vi "VIH Project Tree - Add Files.vi"(6 "Ena dialog message (F)":bool, 8 "error in":errorcluster, 9 "File Paths":path[](array[path]), 10 "Tree Parent Tag":string, 11 "Project Tree":T1) -> (0 "error out":errorcluster, 1 "Top-level Item Tags":string[](array[string]), 3 "dup Project Tree":T1, 4 "Files already in the tree":path[](array[path]))   [LabVIEW 2014]
doc: "::: VI Helpeks :::\nCopyright (c) 2000-2026 Konstantin Shifershteyn. All rights reserved."
uses:
  VIH Project Tree Typedef - Tree Refnum.ctl
  _VIH HelpGen - Palette.llb/VIH HelpGen Typedef - Palette - Item Info Cluster.ctl
  _VIH HelpGen - Palette.llb/VIH HelpGen Typedef - Palette - Item Type Enum.ctl
panel:
  # "VI Helpeks\nCopyright (c) 2012-2026 Konstantin Shifershteyn"
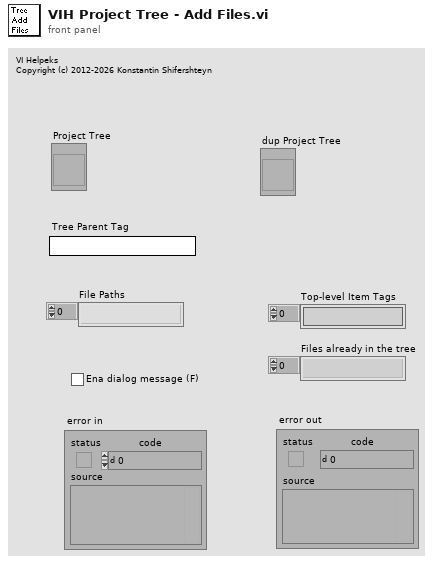
[diagram p1: front panel]
types:
  T1 = typedef "VIH Project Tree Typedef - Tree Refnum.ctl" = refnum<vi>
  T2 = typedef "VIH HelpGen Typedef - Palette - Item Info Cluster.ctl" = cluster{"Item Type":T3, "Item Name":string, "Item File":path, "Parent palette":path, "Not found":bool}
  T3 = typedef "VIH HelpGen Typedef - Palette - Item Type Enum.ctl" = enum32{"<Invalid>", "<unknown>", "VI", "Menu", "LV Func", "Express VI", "Poly VI", "CTL", "HTML"}
  T4 = cluster{"Name":string, "Tag":string, "Child only":bool, "Symbol":i32, "Color":u32}[]
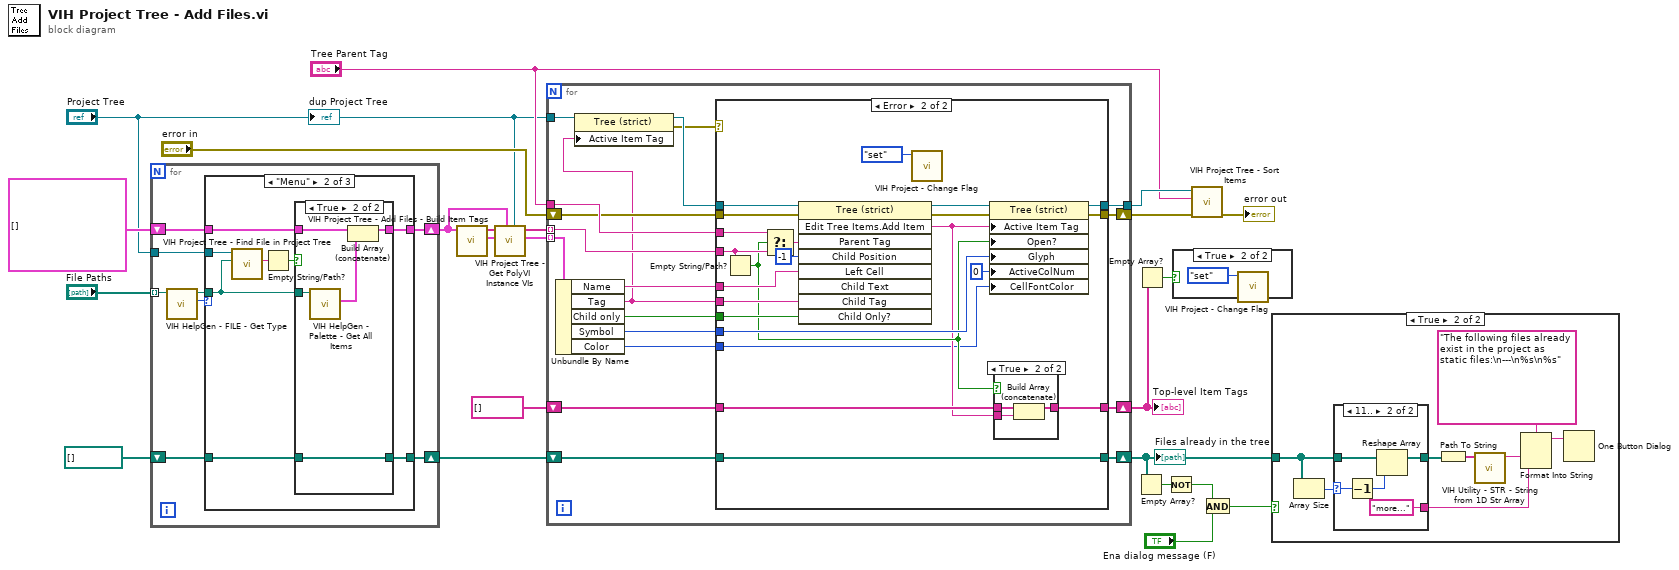
[diagram p0: block diagram]
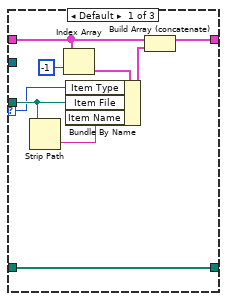
[diagram p2: hidden frame]
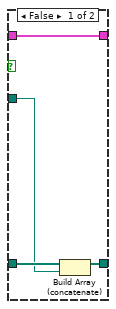
[diagram p3: hidden frame]
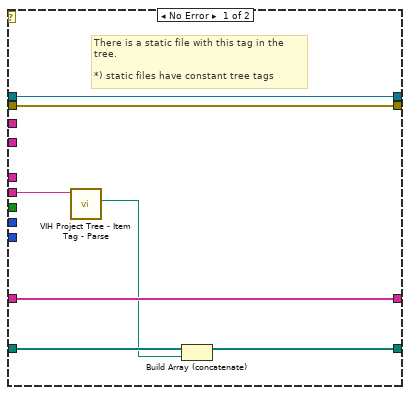
[diagram p8: hidden frame]
diagram:
  n1 = for {
    tunnel: "File Paths" -> [w29] mode=indexing
    shift-right: [w30] -> w4
    shift-left: T2[] [] -> [w31]
    tunnel: "Project Tree" -> [w26]
    shift-right: [w25] -> w2
    shift-left: path[] [] ("Files already in the tree") -> [w24]
    n2 = call "VIH HelpGen - FILE - Get Type.vi"("File Path"=w29) -> ("File Type"=w27:T3, "dup File Path"=w28:path)  [unwired: 8 in, 1 out]
    n3 = case shown="\"Menu\"" w27 {
      selector: w27 -> [w33 _ _]
      tunnel: w28 -> [w39 w46 _]
      tunnel: w31 -> [w35 w48 w59]
      tunnel: [w34 w47 w59] -> w30
      tunnel: w26 -> [_ w45 _]
      tunnel: [w32 w42 w58] -> w25
      tunnel: w24 -> [w32 w41 w58]
      frame Default {
        n4 = Strip Path(path=w39) -> (name=w40:string)  [unwired: 1 out]
        n5 = Index Array(array=w35, index=-1) -> (element=w36:T2)
        n6 = Bundle By Name(cluster=w36, "Item Type"=w33, "Item File"=w39, "Item Name"=w40) -> (w37:T2)
        n7 = Build Array (concatenate)(w35, w37) -> (w34:T2[])
      }
      frame "Menu" {
        n8 = call "VIH Project Tree - Find File in Project Tree.vi"("File Path"=w46, "Project Tree"=w45) -> ("Tree Item Tag (Static)"=w44:string)  [unwired: 6 in, 3 out]
        n9 = Empty String/Path?(string/path=w44) -> (empty?=w43:bool)
        n10 = case shown="True" w43 {
          tunnel: w46 -> [w49 w57]
          tunnel: w48 -> [w52 w56]
          tunnel: [w52 w54] -> w47
          tunnel: [w50 w53] -> w42
          tunnel: w41 -> [w51 w53]
          frame False {
            n11 = Build Array (concatenate)(w51, w49) -> (w50:path[])
          }
          frame True {
            n12 = call "VIH HelpGen - Palette - Get All Items.vi"("Palette Path"=w57) -> ("Items Array"=w55:T2[])  [unwired: 8 in, 2 out]
            n13 = Build Array (concatenate)(w56, w55) -> (w54:T2[])
          }
        }
      }
      frame "LV Func" {
      }
    }
  }
  n14 = call "VIH Project Tree - Add Files - Build Item Tags.vi"("Items Array"=w4) -> ("Item Items Data"=w7:T4, "Item Parent Tags"=w8:string[])  [unwired: 9 in]
  n15 = call "VIH Project Tree - Get PolyVI Instance VIs.vi"("Project Tree"="Project Tree", "Items Array"=w4, "Item Items Data"=w7, "Item Parent Tags"=w8) -> ("Item Items Data out"=w5:T4, "Item Parent Tags out"=w6:string[])  [unwired: 5 in, 1 out]
  n16 = for {
    tunnel: "Project Tree" -> [w66]
    tunnel: [w76] -> w14
    tunnel: "Tree Parent Tag" -> [w77]
    shift-right: [w75] -> w13
    shift-left: "error in" -> [w74]
    tunnel: w6 -> [w73] mode=indexing
    tunnel: w5 -> [w72] mode=indexing
    shift-right: [w67] -> w10
    shift-left: string[] [] ("Top-level Item Tags") -> [w69]
    shift-right: [w62] -> w19
    shift-left: w2 -> [w61]
    n17 = Unbundle By Name(w72) -> ("Name"=w68:string, "Tag"=w64:string, "Child only"=w71:bool, "Symbol"=w70:i32, "Color"=w60:u32)
    n18 = property class="Tree (strict)"(reference=w66, "Active Item Tag"=w64) -> (reference out=w65:T1, error out=w63:errorcluster)  [unwired: 1 in]
    n19 = case shown="Error" w63 {
      tunnel: w77 -> [_ w104]
      tunnel: [w83 w101] -> w76
      tunnel: [w84 w100] -> w75
      tunnel: w74 -> [w84 w99]
      tunnel: w73 -> [_ w97]
      tunnel: w64 -> [w79 w96]
      tunnel: w71 -> [_ w95]
      tunnel: w70 -> [_ w94]
      tunnel: w69 -> [w82 w93]
      tunnel: w68 -> [_ w92]
      tunnel: [w82 w91] -> w67
      tunnel: w65 -> [w83 w88]
      tunnel: [w80 w87] -> w62
      tunnel: w61 -> [w81 w87]
      tunnel: w60 -> [_ w86]
      frame No Error {
        # "There is a static file with this tag in the tree.\n\n*) static files have constant tree tags"
        n20 = call "VIH Project Tree - Item Tag - Parse.vi"("Tree Item Tag"=w79) -> ("Item File Path"=w78:path)  [unwired: 8 in, 2 out]
        n21 = Build Array (concatenate)(w81, w78) -> (w80:path[])
      }
      frame Error {
        n22 = Empty String/Path?(string/path=w97) -> (empty?=w90:bool)
        n23 = Select(t=w104, s=w90, f=w97) -> (s? t:f=w106:string)
        n24 = invoke on="Invoke Node" class="Tree (strict)" method="Edit Tree Items.Add Item"(reference=w88, error in=w99, "Parent Tag"=w106, "Child Position"=-1, "Left Cell"=w92, "Child Tag"=w96, "Child Only?"=w95) -> (reference out=w103:T1, error out=w102:errorcluster, "Edit Tree Items:Add Item"=w89:string)  [unwired: 2 in, 6 out]
        n25 = call "VIH Project - Change Flag.vi"("cmd (get)"=enum16{"get", "set", "reset"}."set") -> ()  [unwired: 9 in, 2 out]
        n26 = property class="Tree (strict)"(reference=w103, error in=w102, "Active Item Tag"=w89, "Open?"=w90, "Glyph"=w94, "ActiveColNum"=0 ("Active Cell:Active Column Number"), "CellFontColor"=w86) -> (reference out=w101:T1, error out=w100:errorcluster)
        n27 = case shown="True" w90 {
          tunnel: w93 -> [w107 w110]
          tunnel: w89 -> [_ w109]
          tunnel: [w107 w108] -> w91
          frame False {
          }
          frame True {
            n28 = Build Array (concatenate)(w110, w109) -> (w108:string[])
          }
        }
      }
    }
  }
  "Top-level Item Tags" <- w10
  "Files already in the tree" <- w19
  n29 = Empty Array?(array=w19) -> (empty?=w18:bool)
  n30 = Empty Array?(array=w10) -> (empty?=w9:bool)
  n31 = Not(x=w18) -> (.not. x?=w17:bool)
  n32 = case shown="True" w9 {
    frame False {
    }
    frame True {
      n33 = call "VIH Project - Change Flag.vi"("cmd (get)"=enum16{"get", "set", "reset"}."set") -> ()  [unwired: 9 in, 2 out]
    }
  }
  n34 = call "VIH Project Tree - Sort Items.vi"("error in"=w13, "Parent Tag"="Tree Parent Tag", "Project Tree"=w14) -> ("error out"=→"error out":errorcluster)  [unwired: 6 in, 2 out]
  n35 = And(x=w17, y="Ena dialog message (F)") -> (x .and. y?=w16:bool)
  n36 = case shown="True" w16 {
    tunnel: w19 -> [_ w113]
    frame False {
    }
    frame True {
      n37 = Array Size(array=w113) -> (size(s)=w115:i32)
      n38 = case shown="11.." w115 {
        selector: w115 -> [_ w123]
        tunnel: [w120 w124] -> w114
        tunnel: w113 -> [w120 w125]
        tunnel: [_ "more..."] -> w112
        frame ..10 {
        }
        frame 11.. {
          n39 = Decrement(x=w123) -> (x-1=w122:i32)
          n40 = Reshape Array(w125, w122) -> (w124:path[])
        }
      }
      n41 = Path To String(path=w114) -> (string=w118:string[])
      n42 = call "VIH Utility - STR - String from 1D Str Array.vi"("Array in"=w118) -> ("String out"=w117:string)  [unwired: 6 in]
      n43 = Format Into String(format string="The following files already exist in the project as static files:\n---\n%s\n%s", w117, w112) -> (resulting string=w116:string)  [unwired: 2 in, 1 out]
      n44 = One Button Dialog(message=w116) -> ()  [unwired: 1 in, 1 out]
    }
  }
  "dup Project Tree" <- "Project Tree"
